vi "TCP Listener.vi"(8 "포트":u16, 9 "네트워크 주소":u32, 11 "Queue Ref":T1) -> ()   [LabVIEW 2023]
uses:
  TCP Socket/TCP Socket.lvclass
panel:
  out "error out":errorcluster
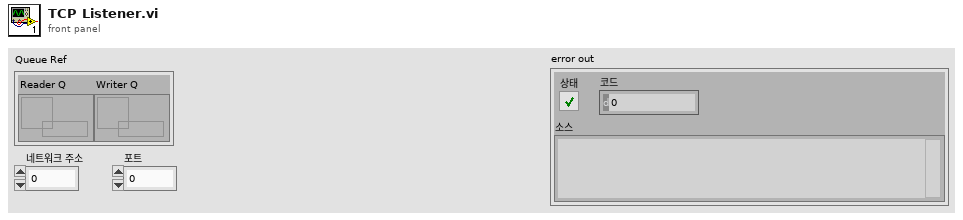
[diagram p1: front panel]
types:
  T1 = cluster{"Reader Q":refnum<queue>, "Writer Q":refnum<queue>}
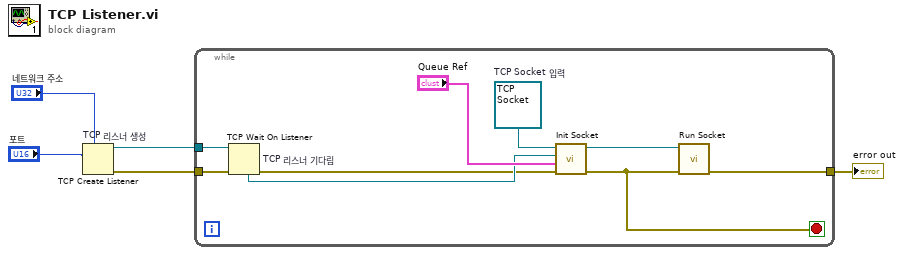
[diagram p0: block diagram]
diagram:
  n1 = TCP Create Listener "TCP 리스너 생성"(7:"네트워크 주소", 10:"포트") -> (0:w4:errorcluster, 3:w5:refnum<k5>)  [unwired: 3 in, 1 out]
  n2 = while {
    tunnel: w5 -> [w14]
    tunnel: w4 -> [w13]
    tunnel: [w10] -> w1
    stop <- w6 stop-if-true
    w9 = refnum<class "TCP Socket.lvclass"> refnum  # TCP Socket 입력
    n3 = TCP Wait On Listener "TCP 리스너 기다림"(8:w13, 11:w14) -> (0:w7:errorcluster, 4:w8:refnum<k5>)  [unwired: 2 in, 3 out]
    n4 = call "Init Socket.vi"("error in (no error)"=w7, "Queue Ref"="Queue Ref", "연결 ID"=w8, "TCP Socket 입력"=w9) -> ("error out"=w6:errorcluster, "TCP Socket 출력"=w12:refnum<class "TCP Socket.lvclass">)  [unwired: 6 in]
    n5 = call "Run Socket.vi"("error in (no error)"=w6, "TCP Socket 입력"=w12) -> ("error out"=w10:errorcluster)  [unwired: 8 in, 1 out]
  }
  "error out" <- w1
